vi "DSS-test-lin_calc_impedance.vi"(8 "error in":errorcluster) -> (0 "error out":errorcluster)   [LabVIEW 2020, in "DSS-Tests.lvlib"]
doc: "Caraya test of RDC-Lin-Calc_Impedance for the reflections 0, 0.5, -0.5 and 0.3+0.4i: Impedance and Admittance against their golden file, and Impedance against Z = 50(1+G)/(1-G) computed here."
uses:
  DSS-Tests.lvlib
  <vilib>/addons/_JKI Toolkits/Caraya/classes/Test/Test.lvclass
  Computation/RDC-Reflection_Data_Computation.lvlib
  <vilib>/addons/_JKI Toolkits/Caraya/classes/Assert/Assert.lvclass
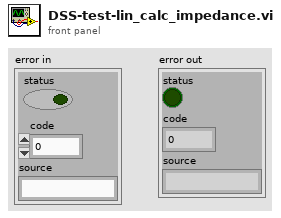
[diagram p1: front panel]
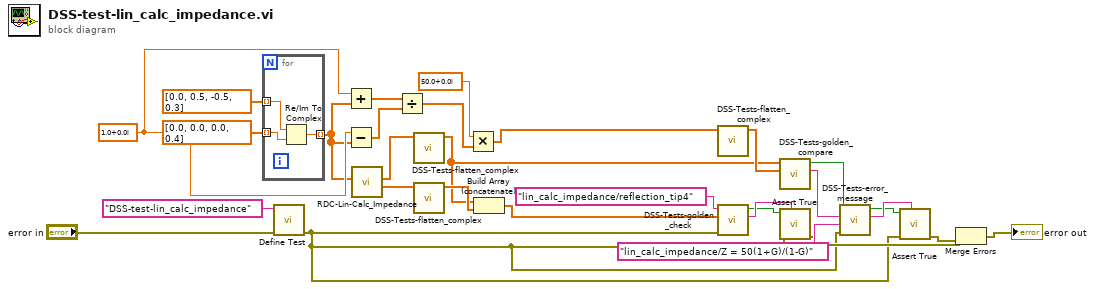
[diagram p0: block diagram]
diagram:
  w16 = cdb 1.0+0.0i ("one")
  n1 = for {
    tunnel: dbl[] [0.0, 0.5, -0.5, 0.3] ("reflection re") -> [w30] mode=indexing
    tunnel: dbl[] [0.0, 0.0, 0.0, 0.4] ("reflection im") -> [w31] mode=indexing
    tunnel: [w32] -> w6 mode=indexing
    n2 = Re/Im To Complex(1:w31, 2:w30) -> (0:w32:cdb)
  }
  n3 = call <vilib>:"Define Test.vi"("error in (no error)"="error in", "Label (VI Title)"="DSS-test-lin_calc_impedance") -> ("error out"=w3:errorcluster)  [unwired: 8 in, 1 out]
  n4 = Add(x=w16, y=w6) -> (x+y=w18:cdb[])
  n5 = Subtract(x=w16, y=w6) -> (x-y=w19:cdb[])
  n6 = call "RDC-Lin-Calc_Impedance.vi"("Reflection Tip"=w6) -> ("Admittance"=w8:cdb[], "Impedance"=w7:cdb[])  [unwired: 9 in]
  n7 = Divide(x=w18, y=w19) -> (x/y=w20:cdb[])
  n8 = call "DSS-Tests-flatten_complex.vi"("values"=w7) -> ("flat"=w9:dbl[])  [unwired: 10 in]
  n9 = call "DSS-Tests-flatten_complex.vi"("values"=w8) -> ("flat"=w10:dbl[])  [unwired: 10 in]
  n10 = Multiply(x=cdb 50.0+0.0i ("Z0"), y=w20) -> (x*y=w21:cdb[])
  n11 = Build Array (concatenate)(w9, w10) -> (w11:dbl[])
  n12 = call "DSS-Tests-flatten_complex.vi"("values"=w21) -> ("flat"=w22:dbl[])  [unwired: 10 in]
  n13 = call "DSS-Tests-golden_check.vi"("error in"=w3, "actual"=w11, "golden name"="lin_calc_impedance/reflection_tip4") -> ("message"=w14:string, "pass"=w13:bool)  [unwired: 6 in, 1 out]
  n14 = call "DSS-Tests-golden_compare.vi"("golden"=w22, "actual"=w9) -> ("message"=w24:string, "pass"=w23:bool)  [unwired: 7 in, 1 out]
  n15 = call <vilib>:"Assert True.vi"("Label"=w14, "error in (no error)"=w3, "True?"=w13) -> ("error out"=w15:errorcluster)  [unwired: 7 in, 1 out]
  n16 = call "DSS-Tests-error_message.vi"("error in"=w3, "prefix"="lin_calc_impedance/Z = 50(1+G)/(1-G)", "message in"=w24, "pass in"=w23) -> ("message"=w27:string, "pass"=w26:bool)  [unwired: 5 in, 1 out]
  n17 = call <vilib>:"Assert True.vi"("Label"=w27, "error in (no error)"=w3, "True?"=w26) -> ("error out"=w28:errorcluster)  [unwired: 7 in, 1 out]
  n18 = Merge Errors(w15, w28) -> (→"error out":errorcluster)
